vi "DAQmx config to DAQ config (AO and AI).vi"(8 "error in (no error)":errorcluster, 10 "AO config":T1 {"output terminal configuration" items=[""=-1, "Differential"=10106, "Pseudodifferential"=12529]}, 11 "AI config":T4 {"input terminal configuration" items=[""=-1, "Differential"=10106, "Pseudodifferential"=12529]; "Coupling" items=["AC"=10045, "DC"=10050, "GND"=10066]}) -> (0 "error out":errorcluster, 2 "AO Config":T13, 3 "AI Config":T8)   [LabVIEW 2019, in "Instrument.Lockin.lvlib" / "Instrument.DAQ.lvclass"]
uses:
  Instrument.DAQ.lvclass
  Lockin.Typedefs/DAQ/DAQ.Config.AO--Cluster--Array.ctl
  Lockin.Typedefs/DAQ/DAQ.Config.AO--Cluster.ctl
  Lockin.Typedefs/DAQ/DAQ.Config.AO.Range--enum.ctl
  Lockin.Typedefs/DAQ/DAQ.TerminalConfiguration--enum.ctl
  Lockin.Typedefs/DAQ/DAQ.Config.AI--Cluster--Array.ctl
  Lockin.Typedefs/DAQ/DAQ.Config.AI--Cluster.ctl
  Lockin.Typedefs/DAQ/DAQ.Config.AI.Coupling--enum.ctl
  Lockin.Typedefs/DAQ/DAQ.Config.AI.Range--enum.ctl
  Lockin.Typedefs/Lockin.Typedefs.lvlib
  DAQmx/typedefs/DAQmx.Config.AI.Coupling--enum.ctl
  DAQmx/DAQmx.lvclass
  DAQmx/typedefs/DAQmx.Config.AI.Range--enum.ctl
  DAQmx/typedefs/DAQmx.Config.AI--Cluster.ctl
  DAQmx/typedefs/DAQmx.Config.AI--Cluster--Array.ctl
  DAQmx/typedefs/DAQmx.Config.AO.Range--enum.ctl
  DAQmx/typedefs/DAQmx.Config.AO--Cluster.ctl
  DAQmx/typedefs/DAQmx.Config.AO--Cluster--Array.ctl
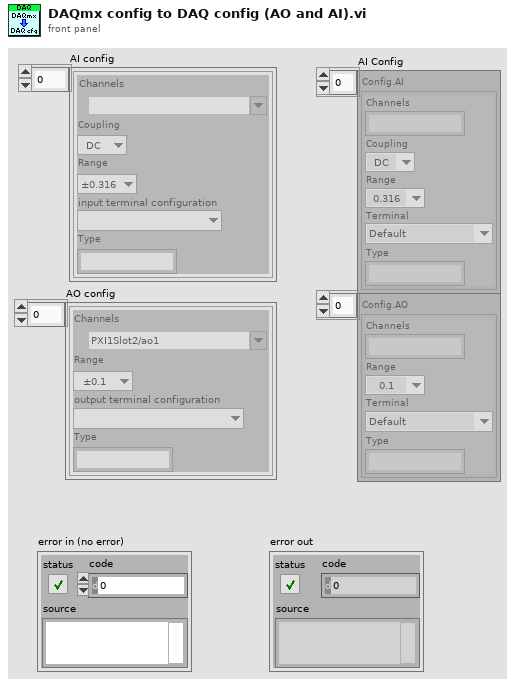
[diagram p1: front panel]
types:
  T1 = typedef "DAQmx.lvclass/DAQmx.Config.AO--Cluster--Array.ctl" = T2[]
  T2 = typedef "DAQmx.lvclass/DAQmx.Config.AO--Cluster.ctl" = cluster{"Channels":tag, "Range":T3, "output terminal configuration":i32, "Type":string}
  T3 = typedef "DAQmx.lvclass/DAQmx.Config.AO.Range--enum.ctl" = enum16{"±0.1", "±1.0", "±3.5", "±10.0"}
  T4 = typedef "DAQmx.lvclass/DAQmx.Config.AI--Cluster--Array.ctl" = T5[]
  T5 = typedef "DAQmx.lvclass/DAQmx.Config.AI--Cluster.ctl" = cluster{"Channels":tag, "Coupling":T6, "Range":T7, "input terminal configuration":i32, "Type":string}
  T6 = typedef "DAQmx.lvclass/DAQmx.Config.AI.Coupling--enum.ctl" = u16
  T7 = typedef "DAQmx.lvclass/DAQmx.Config.AI.Range--enum.ctl" = enum16{"±0.316", "±1.00", "±3.16", "±10.0", "±31.6", "±42.4"}
  T8 = typedef "Lockin.Typedefs.lvlib/DAQ.Config.AI--Cluster--Array.ctl" = T9[]
  T9 = typedef "Lockin.Typedefs.lvlib/DAQ.Config.AI--Cluster.ctl" = cluster{"Channels":string, "Coupling":T10, "Range":T11, "Terminal":T12, "Type":string}
  T10 = typedef "Lockin.Typedefs.lvlib/DAQ.Config.AI.Coupling--enum.ctl" = enum16{"AC", "DC", "GND", ""}
  T11 = typedef "Lockin.Typedefs.lvlib/DAQ.Config.AI.Range--enum.ctl" = enum16{"0.316", "1.00", "3.16", "10.0", "31.6", "42.4", ""}
  T12 = typedef "Lockin.Typedefs.lvlib/DAQ.TerminalConfiguration--enum.ctl" = enum16{"Default", "Differential", "Pseudodifferential", ""}
  T13 = typedef "Lockin.Typedefs.lvlib/DAQ.Config.AO--Cluster--Array.ctl" = T14[]
  T14 = typedef "Lockin.Typedefs.lvlib/DAQ.Config.AO--Cluster.ctl" = cluster{"Channels":string, "Range":T15, "Terminal":T12, "Type":string}
  T15 = typedef "Lockin.Typedefs.lvlib/DAQ.Config.AO.Range--enum.ctl" = enum16{"0.1", "1.0", "3.5", "10.0", ""}
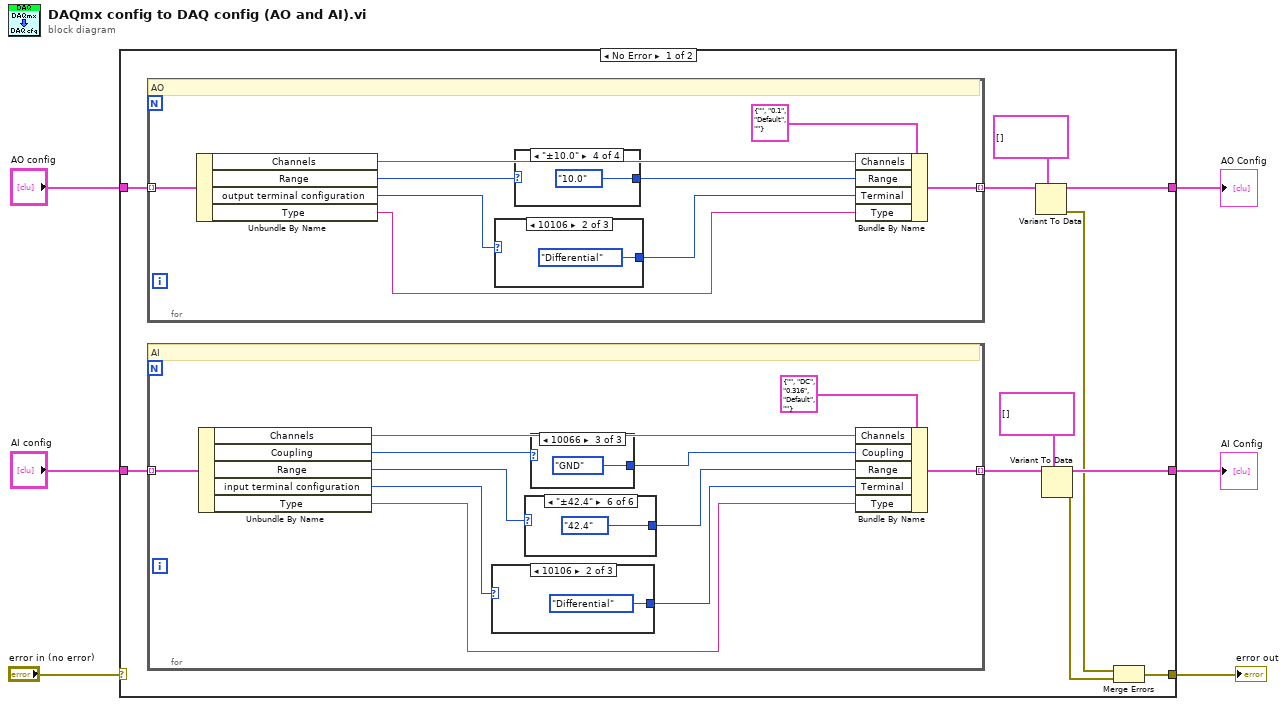
[diagram p0: block diagram]
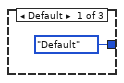
[diagram p2: hidden frame]
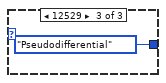
[diagram p3: hidden frame]
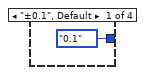
[diagram p4: hidden frame]
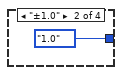
[diagram p5: hidden frame]
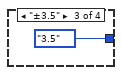
[diagram p6: hidden frame]
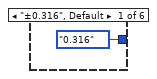
[diagram p7: hidden frame]
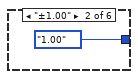
[diagram p8: hidden frame]
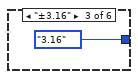
[diagram p9: hidden frame]
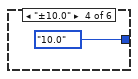
[diagram p10: hidden frame]
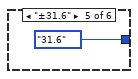
[diagram p11: hidden frame]
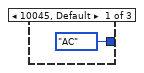
[diagram p12: hidden frame]
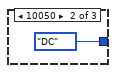
[diagram p13: hidden frame]
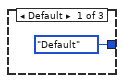
[diagram p14: hidden frame]
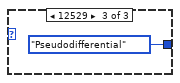
[diagram p15: hidden frame]
diagram:
  n1 = case shown="No Error" "error in (no error)" {
    selector: "error in (no error)" -> [_ w57]
    tunnel: "AO config" -> [w16 _]
    tunnel: [w9 w57] -> w5
    tunnel: "AI config" -> [w17 _]
    tunnel: [w13 _] -> w3
    tunnel: [w12 _] -> w4
    frame No Error {
      n2 = for {
        tunnel: w16 -> [w26] mode=indexing
        tunnel: [w25] -> w14 mode=indexing
        # "AO"
        n3 = Unbundle By Name(w26) -> ("Channels"=w23:tag, "Range"=w19:T3, "output terminal configuration"=w18:i32, "Type"=w24:string)
        n4 = case shown="10106" w18 {
          tunnel: [DAQ.TerminalConfiguration--enum."Default" ("Terminal") DAQ.TerminalConfiguration--enum."Differential" ("Terminal") DAQ.TerminalConfiguration--enum."Pseudodifferential" ("Terminal")] -> w21
          frame Default {
          }
          frame 10106 {
          }
          frame 12529 {
          }
        }
        n5 = case shown="\"±10.0\"" w19 {
          tunnel: [DAQ.Config.AO.Range--enum."0.1" ("Range") DAQ.Config.AO.Range--enum."1.0" ("Range") DAQ.Config.AO.Range--enum."3.5" ("Range") DAQ.Config.AO.Range--enum."10.0" ("Range")] -> w22
          frame "±0.1", Default {
          }
          frame "±1.0" {
          }
          frame "±3.5" {
          }
          frame "±10.0" {
          }
        }
        n6 = Bundle By Name(cluster=T14 {"Channels"="", "Range"=enum."0.1", "Terminal"=enum."Default", "Type"=""} ("Config.AO"), "Channels"=w23, "Range"=w22, "Terminal"=w21, "Type"=w24) -> (w25:T14)
      }
      n7 = for {
        tunnel: [w44] -> w15 mode=indexing
        tunnel: w17 -> [w43] mode=indexing
        # "AI"
        n8 = Unbundle By Name(w43) -> ("Channels"=w42:tag, "Coupling"=w36:T6, "Range"=w34:T7, "input terminal configuration"=w38:i32, "Type"=w41:string)
        n9 = case shown="10106" w38 {
          tunnel: [DAQ.TerminalConfiguration--enum."Default" ("Terminal") DAQ.TerminalConfiguration--enum."Differential" ("Terminal") DAQ.TerminalConfiguration--enum."Pseudodifferential" ("Terminal")] -> w37
          frame Default {
          }
          frame 10106 {
          }
          frame 12529 {
          }
        }
        n10 = case shown="\"±42.4\"" w34 {
          tunnel: [DAQ.Config.AI.Range--enum."0.316" ("Range") DAQ.Config.AI.Range--enum."1.00" ("Range") DAQ.Config.AI.Range--enum."3.16" ("Range") DAQ.Config.AI.Range--enum."10.0" ("Range") DAQ.Config.AI.Range--enum."31.6" ("Range") DAQ.Config.AI.Range--enum."42.4" ("Range")] -> w35
          frame "±0.316", Default {
          }
          frame "±1.00" {
          }
          frame "±3.16" {
          }
          frame "±10.0" {
          }
          frame "±31.6" {
          }
          frame "±42.4" {
          }
        }
        n11 = case shown="10066" w36 {
          tunnel: [DAQ.Config.AI.Coupling--enum."AC" ("Coupling") DAQ.Config.AI.Coupling--enum."DC" ("Coupling") DAQ.Config.AI.Coupling--enum."GND" ("Coupling")] -> w39
          frame 10045, Default {
          }
          frame 10050 {
          }
          frame 10066 {
          }
        }
        n12 = Bundle By Name(cluster=T9 {"Channels"="", "Coupling"=enum."DC", "Range"=enum."0.316", "Terminal"=enum."Default", "Type"=""} ("Config.AI"), "Channels"=w42, "Coupling"=w39, "Range"=w35, "Terminal"=w37, "Type"=w41) -> (w44:T9)
      }
      n13 = Variant To Data(type=T13 [] ("AO Config"), Variant=w14) -> (data=w12:T13, error out=w11:errorcluster)  [unwired: 1 in]
      n14 = Variant To Data(type=T8 [] ("AI Config"), Variant=w15) -> (data=w13:T8, error out=w10:errorcluster)  [unwired: 1 in]
      n15 = Merge Errors(w11, w10) -> (w9:errorcluster)
    }
    frame Error {
    }
  }
  "AO Config" <- w4
  "error out" <- w5
  "AI Config" <- w3
